vi "Actor Core.vi"(8 "error in":errorcluster, 11 "Nested in":refnum<class "ChannelManagerUI.lvclass">) -> (0 "error out":errorcluster, 3 "Actor out":refnum<class "Actor.lvclass">)   [LabVIEW 2021, in "Channel.lvlib" / "ChannelManagerUI.lvlib" / "ChannelManagerUI.lvclass"]
doc: "(<B>Filename</B>: Actor Framework.lvlib:Actor.lvclass:Actor Core.vi)\n\nReceives messages to the actor, reacts to them, and initiates any error handling that may shut the actor down.\n\nDescendant classes may override this VI to append parallel tasks for the actor to complete while it handles messages. Overrides use the Call Parent Method node."
uses:
  ChannelManagerUI.lvclass
  C:/Program Files/National Instruments/LabVIEW 2021/vi.lib/ActorFramework/Actor/Actor.lvclass
  <vilib>/ActorFramework/Actor/Actor.lvclass
  tdef/UI-References.ctl
  tdef/UI-Refs-SideButtons.ctl
  ChannelManagerUI.lvclass/ChannelManagerUI.ctl
  <vilib>/ActorFramework/Actor/Actor.lvclass/Actor.ctl
  <vilib>/ActorFramework/Message Enqueuer/Message Enqueuer.lvclass/Message Enqueuer.ctl
  ChannelsManager/ChannelsManager Messages/RemoveChannel Msg/RemoveChannel Msg.lvclass/RemoveChannel Msg.ctl
  Messages/SetSelectedChannel_Msg/SetSelectedChannel_Msg.lvclass/SetSelectedChannel_Msg.ctl
  <vilib>/ActorFramework/Message Enqueuer/Init from Existing Queue.vi
  <vilib>/ActorFramework/Message Enqueuer/Enqueue.vi
  ChannelManagerUI Messages/Timeout Msg/Timeout Msg.lvclass
  C:/Program Files/National Instruments/LabVIEW 2021/vi.lib/ActorFramework/Message/Message.lvclass
  <vilib>/ActorFramework/Stop Msg/Stop Msg.lvclass
  ChannelManagerUI Messages/New Channel Msg/New Channel Msg.lvclass
  ChannelsManager/ChannelsManager Messages/RemoveChannel Msg/RemoveChannel Msg.lvclass
  ChannelsManager/ChannelsManager Messages/SaveChannels Msg/SaveChannels Msg.lvclass
  ChannelManagerUI Messages/Edit Channel Msg/Edit Channel Msg.lvclass
  Messages/SetSelectedChannel_Msg/SetSelectedChannel_Msg.lvclass
  <vilib>/ActorFramework/Message Priority Queue/Priority Enqueue.vi
  <vilib>/ActorFramework/Message Enqueuer/Message Enqueuer.lvclass
  ChannelsManager/ChannelsManager/ChannelsManager.lvclass
  ChannelManagerUI Messages/Load Plugins Msg/Load Plugins Msg.lvclass
  C:/Users/averna/Documents/LV Gym DEMO/Factory Pattern/Generic Channel/Channel/ChannelsManager/ChannelsManager/ChannelsManager.lvclass
  C:/Users/averna/Documents/LV Gym DEMO/Factory Pattern/Generic Channel/Channel/ChannelManagerUI/ChannelManagerUI.lvclass
  Channel.lvlib
panel:
  in  "Channels Name":i32(listbox)
  out "Configuration":path
  out "Plugns Folder":path
  out "Channel Type":string
  in  "Load Plugins":bool
  in  "Edit":bool
  in  "Save":bool
  in  "Reload":bool
  in  "Remove Channel":bool
  in  "New Channel":bool
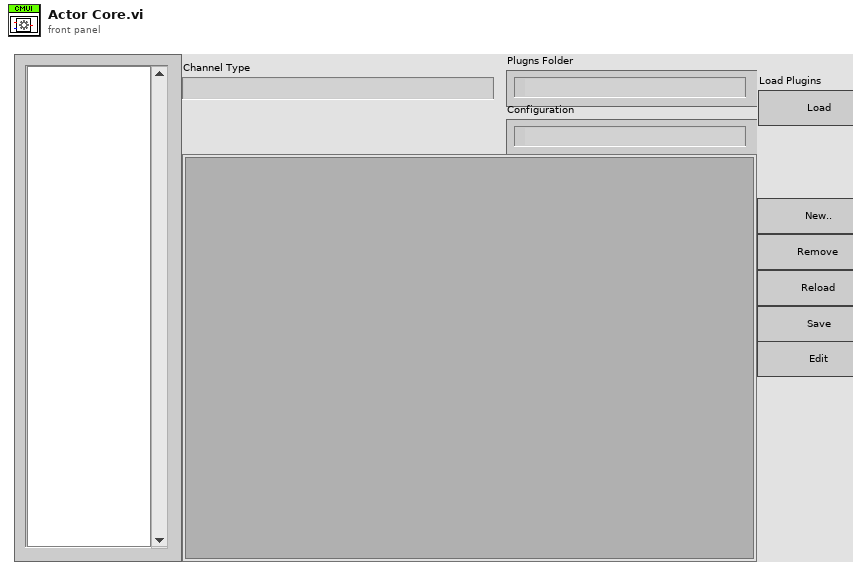
[diagram p1: front panel]
types:
  T1 = typedef "Channel.lvlib/ChannelManagerUI.lvlib/ChannelManagerUI.lvclass/UI-References.ctl" = cluster{"Side Buttons":T2, "Sub Panel":refnum<vi>}
  T2 = typedef "Channel.lvlib/ChannelManagerUI.lvlib/ChannelManagerUI.lvclass/UI-Refs-SideButtons.ctl" = cluster{"New":refnum<vi>, "Remove":refnum<vi>, "Reload":refnum<vi>, "Save":refnum<vi>, "Edit":refnum<vi>}
  T3 = cluster{"Stop":refnum<user-event>, "Channels List":refnum<user-event>, "Channel Type":refnum<user-event>}
  T4 = enum8{"Enabled", "Disabled", "Disabled and Grayed Out"}
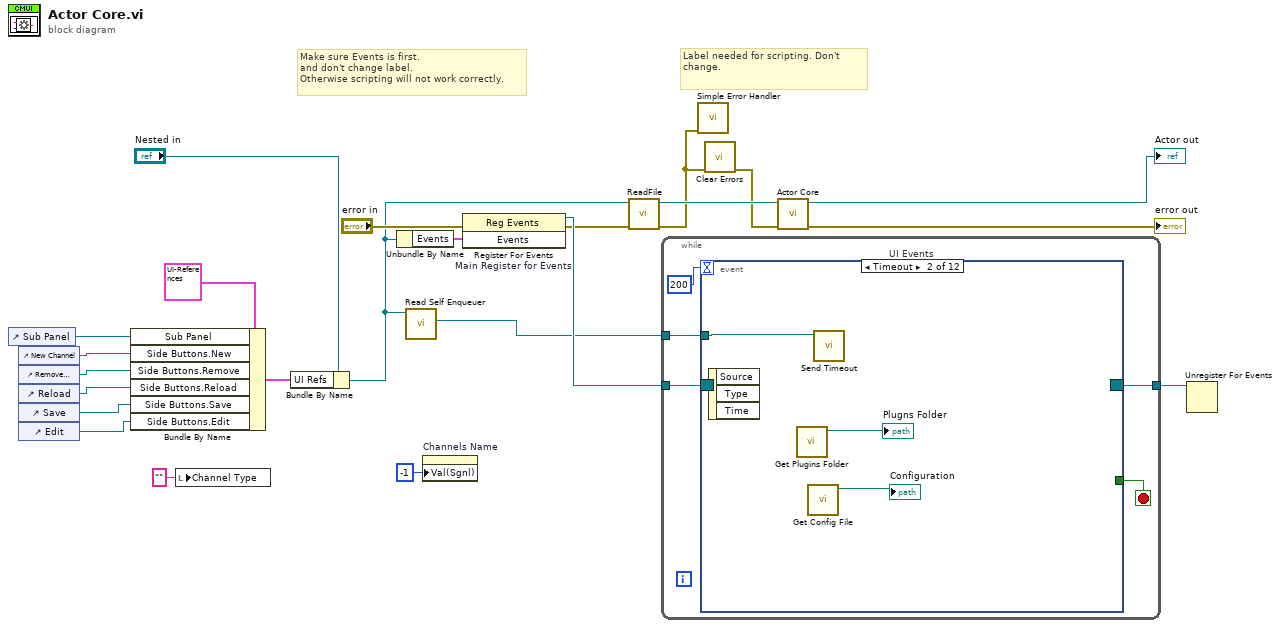
[diagram p0: block diagram]
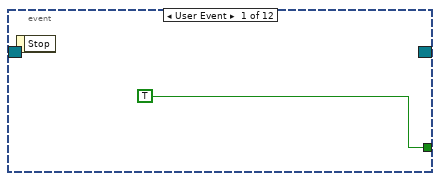
[diagram p2: hidden frame]
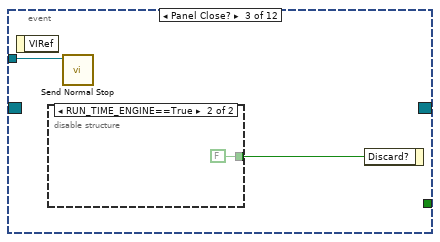
[diagram p3: hidden frame]
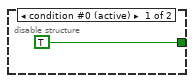
[diagram p4: hidden frame]
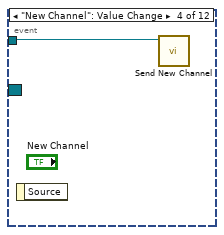
[diagram p5: hidden frame]
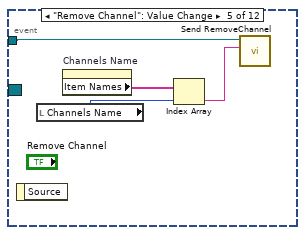
[diagram p6: hidden frame]
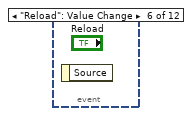
[diagram p7: hidden frame]
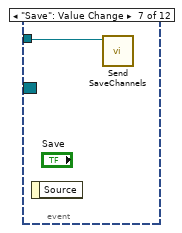
[diagram p8: hidden frame]
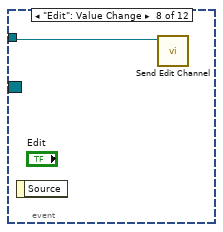
[diagram p9: hidden frame]
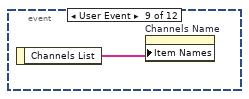
[diagram p10: hidden frame]
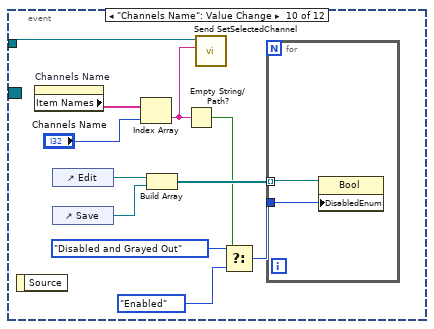
[diagram p11: hidden frame]
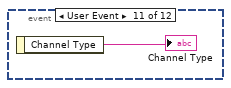
[diagram p12: hidden frame]
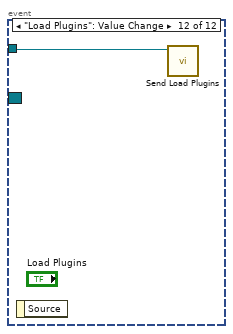
[diagram p13: hidden frame]
diagram:
  # "Label needed for scripting. Don't change."
  # "Make sure Events is first.\nand don't change label.\nOtherwise scripting will not work correctly."
  n1 = control-ref of="Sub Panel"() -> (w16:refnum<vi>)
  n2 = control-ref of="New Channel"() -> (w12:refnum<vi>)
  n3 = control-ref of="Remove Channel"() -> (w11:refnum<vi>)
  n4 = control-ref of="Reload"() -> (w10:refnum<vi>)
  n5 = control-ref of="Save"() -> (w9:refnum<vi>)
  n6 = control-ref of="Edit"() -> (w8:refnum<vi>)
  n7 = Bundle By Name(cluster=T1 {"Side Buttons"={"New"=refnum, "Remove"=refnum, "Reload"=refnum, "Save"=refnum, "Edit"=refnum}, "Sub Panel"=refnum} ("UI Refs"), "Sub Panel"=w16, "Side Buttons.New"=w12, "Side Buttons.Remove"=w11, "Side Buttons.Reload"=w10, "Side Buttons.Save"=w9, "Side Buttons.Edit"=w8) -> (w13:T1)
  n8 = local write "Channel Type"("" ("Channel Type")) -> ()
  n9 = Bundle By Name(cluster="Nested in", "UI Refs"=w13) -> (w14:refnum<class "ChannelManagerUI.lvclass">)
  n10 = Unbundle By Name(w14) -> ("Events"=w6:T3)
  n11 = call <vilib>:"Read Self Enqueuer.vi"("Actor"=w14) -> ("Self Enqueuer"=w19:refnum<class "Message Enqueuer.lvclass">)  [unwired: 10 in]
  n12 = property on="Channels Name" class="LstBox (strict)"("Val(Sgnl)"=-1 ("Value (Signaling)")) -> ()  [unwired: 2 in, 2 out]
  n13 = register-events "Main Register for Events"(error in="error in", w6) -> (reference out=w21:refnum<event-registration>, error out=w5:errorcluster)  [unwired: 1 in]
  n14 = call-dynamic "ReadFile.vi"("error in (no error)"=w5, "object in"=w14) -> ("error out"=w1:errorcluster, "object out"=w7:refnum<class "ChannelManagerUI.lvclass">)  [unwired: 8 in]
  n15 = while {
    tunnel: w21 -> [w28]
    tunnel: [w26] -> w20
    tunnel: w19 -> [w25]
    stop <- w27 stop-if-true
    n16 = event "UI Events" shown="[1] Timeout" {
      selector: w28 -> [_ _ _ _ _ _ _ _ _ _ _ _]
      dyn-events: [_ _ _ _ _ _ _ _ _ _ _ _] -> w26
      timeout: 200 -> [_ _ _ _ _ _ _ _ _ _ _ _]
      tunnel: [TRUE _ _ _ _ _ _ _ _ _ _ _] -> w27
      tunnel: w25 -> [_ w32 w33 w37 w41 _ w42 w43 _ w46 _ w59]
      event User Event {
        n17 = event-data() -> ()  [unwired: 1 in, 1 out]
      }
      event Timeout {
        n18 = event-data() -> ()  [unwired: 1 in, 3 out]
        n19 = call "Get Plugins Folder.vi"() -> ("Plugins Folder"=→"Plugns Folder":path)  [unwired: 10 in, 1 out]
        n20 = call "Get Config File.vi"() -> ("Config File"=→"Configuration":path)  [unwired: 10 in, 1 out]
        n21 = call "Send Timeout.vi"("Message Enqueuer"=w32) -> ()  [unwired: 9 in, 2 out]
      }
      event Panel Close? {
        n22 = event-data() -> ()  [unwired: 1 in, 1 out]
        n23 = disable-structure shown="RUN_TIME_ENGINE==True" {
          disable-tunnel: [TRUE ("Discard?") FALSE ("Discard?")] -> w34
          frame condition #0 (active) {
          }
          frame condition #1 {
          }
        }
        n24 = call <vilib>:"Send Normal Stop.vi"("Message Enqueuer"=w33) -> ()  [unwired: 10 in, 1 out]
        n25 = event-data("Discard?"=w34) -> ()  [unwired: 1 in, 1 out]
      }
      event "New Channel": Value Change {
        n26 = event-data() -> ()  [unwired: 1 in, 1 out]
        n27 = call "Send New Channel.vi"("Message Enqueuer"=w37) -> ()  [unwired: 9 in, 2 out]
      }
      event "Remove Channel": Value Change {
        n28 = event-data() -> ()  [unwired: 1 in, 1 out]
        n29 = local read "Channels Name"() -> (w39:i32)
        n30 = property on="Channels Name" class="LstBox (strict)"() -> ("Item Names"=w40:string[])  [unwired: 2 in, 2 out]
        n31 = Index Array(array=w40, index=w39) -> (element=w38:string)
        n32 = call "Send RemoveChannel.vi"("Name"=w38, "Message Enqueuer"=w41) -> ()  [unwired: 8 in, 2 out]
      }
      event "Reload": Value Change {
        n33 = event-data() -> ()  [unwired: 1 in, 1 out]
      }
      event "Save": Value Change {
        n34 = event-data() -> ()  [unwired: 1 in, 1 out]
        n35 = call "Send SaveChannels.vi"("Message Enqueuer"=w42) -> ()  [unwired: 9 in, 2 out]
      }
      event "Edit": Value Change {
        n36 = event-data() -> ()  [unwired: 1 in, 1 out]
        n37 = call "Send Edit Channel.vi"("Message Enqueuer"=w43) -> ()  [unwired: 9 in, 2 out]
      }
      event User Event {
        n38 = event-data() -> ("Channels List"=w44:string[])  [unwired: 1 in]
        n39 = property on="Channels Name" class="LstBox (strict)"("Item Names"=w44) -> ()  [unwired: 2 in, 2 out]
      }
      event "Channels Name": Value Change {
        n40 = event-data() -> ()  [unwired: 1 in, 1 out]
        n41 = property on="Channels Name" class="LstBox (strict)"() -> ("Item Names"=w55:string[])  [unwired: 2 in, 2 out]
        n42 = control-ref of="Edit"() -> (w53:refnum<vi>)
        n43 = control-ref of="Save"() -> (w52:refnum<vi>)
        n44 = Index Array(array=w55, index="Channels Name") -> (element=w45:string)
        n45 = Build Array(w53, w52) -> (w51:refnum<vi>[])
        n46 = Empty String/Path?(string/path=w45) -> (empty?=w47:bool)
        n47 = call "Send SetSelectedChannel.vi"("Channel Name"=w45, "Message Enqueuer"=w46) -> ()  [unwired: 8 in, 2 out]
        n48 = Select(t=T4."Disabled and Grayed Out", s=w47, f=T4."Enabled" ("Disabled")) -> (s? t:f=w50:T4)
        n49 = for {
          tunnel: w51 -> [w57] mode=indexing
          tunnel: w50 -> [w56]
          n50 = property class="Bool"(reference=w57, "DisabledEnum"=w56) -> ()  [unwired: 1 in, 2 out]
        }
      }
      event User Event {
        n51 = event-data() -> ("Channel Type"=→"Channel Type":string)  [unwired: 1 in]
      }
      event "Load Plugins": Value Change {
        n52 = event-data() -> ()  [unwired: 1 in, 1 out]
        n53 = call "Send Load Plugins.vi"("Message Enqueuer"=w59) -> ()  [unwired: 9 in, 2 out]
      }
    }
  }
  n54 = call <vilib>:"Simple Error Handler.vi"("error in (no error)"=w1) -> ()  [unwired: 4 in, 5 out]
  n55 = call <vilib>:"Clear Errors.vi"("error in (no error)"=w1) -> ("error out"=w2:errorcluster)  [unwired: 5 in, 1 out]
  n56 = call-parent "Actor Core.vi"("error in"=w2, "Actor in"=w7) -> ("error out"=→"error out":errorcluster, "Actor out"=→"Actor out":refnum<class "Actor.lvclass">)  [unwired: 8 in]
  n57 = Unregister For Events(event registration refnum=w20) -> ()  [unwired: 1 in, 1 out]
